vi "Autonomous Independent.vi"   [LabVIEW 2016]
doc: "This VI is called when autonomous begins, and will automatically be terminated when autonomous ends. You can carry out timed or sensor driven robot movement independently without needing to return to the caller."
uses:
  <vilib>/Rock Robotics/WPI/Ultrasonic/WPI_UltrasonicRangeUnits.ctl
  <vilib>/Rock Robotics/WPI/Utilities/WPI_GetSetVariantRefNum.vi
  <vilib>/Rock Robotics/Network Tables/NT Read String.vi
  <vilib>/Rock Robotics/Network Tables/NT Write Numeric Array.vi
  <vilib>/Rock Robotics/WPI/Ultrasonic/WPI_SonarSRF04DigitalRefNum Registry Get.vi
  <vilib>/Rock Robotics/WPI/Ultrasonic/WPI_SonarSRF04DigitalGetRange.vi
panel:
  # "Be sure to right-click and choose Data Operations>>Make Current Value default if you want to save the array values with the VI"
types:
  T1 = typedef "WPI_DriverStationPositionInfo.ctl" = enum16{"1", "2", "3"}
  T2 = typedef "WPI_JoystickDevRef.ctl" = cluster{"Device":T3}
  T3 = typedef "WPI_JoystickDeviceEnum.ctl" = enum16{"USB 0", "USB 1", "USB 2", "USB 3", "USB 4", "USB 5"}
  T4 = typedef "WPI_UltrasonicRangeUnits.ctl" = enum16{"inches", "mm"}
  T5 = typedef "WPI_EncoderDevRef.ctl" = cluster{"DevStatus":errorcluster, "EncoderIndex":T6, "CounterIndex":T7, "DistancePerCount":dbl, "Decoding Type":T8}
  T6 = typedef "FPGA_EncoderIdx.ctl" = enum8{"Enc 0", "Enc 1", "Enc 2", "Enc 3", "Enc 4", "Enc 5", "Enc 6", "Enc 7", "Invalid"}
  T7 = typedef "FPGA_CounterCtrSystemIndex.ctl" = enum8{"Ctr 0", "Ctr 1", "Ctr 2", "Ctr 3", "Ctr 4", "Ctr 5", "Ctr 6", "Ctr 7", "Invalid"}
  T8 = typedef "WPI_EncoderType.ctl" = enum16{"1x", "2x", "4x"}
  T9 = typedef "WPI_RobotDriveDevRef.ctl" = cluster{"DevStatus":errorcluster, "Motors[]":T10[], "Square Inputs":bool, "Max Output":dbl}
  T10 = typedef "WPI_MotorControlDeviceRef.ctl" = cluster{"DeviceStatus":errorcluster, "Type":T11, "PWM":cluster{"PWM Channel":T12, "DeadBand":T13}, "CAN":cluster{"Device Number":u8, "SetOutput VI Ref":variant, "GetOutput VI Ref":variant, "Enable VI Ref":variant, "Disable VI Ref":variant, "Data":variant}, "Invert":bool}
  T11 = typedef "WPI_MotorControlType.ctl" = enum16{"PWM", "CAN"}
  T12 = typedef "FPGA_DIOPWMChannel.ctl" = enum8{"PWM 0", "PWM 1", "PWM 2", "PWM 3", "PWM 4", "PWM 5", "PWM 6", "PWM 7", "PWM 8", "PWM 9", "PWM MXP 0", "PWM MXP 1", "PWM MXP 2", "PWM MXP 3", "PWM MXP 4", "PWM MXP 5", "PWM MXP 6", "PWM MXP 7", "PWM MXP 8", "PWM MXP 9", "Invalid"}
  T13 = typedef "WPI_PWMDeadband.ctl" = cluster{"Name":string, "maxPositivePwm":i32, "minPositivePwm":i32, "centerPwm":i32, "maxNegativePwm":i32, "minNegativePwm":i32, "angularRange":u16}
  T14 = typedef "Image Type" = u32
  T15 = typedef "WPI_CameraDevRef.ctl" = cluster{"Camera Address":string, "CameraStatus":errorcluster}
  T16 = typedef "WPI_CameraImageSize.ctl" = enum16{"640x480", "320x240", "160x120", "Custom"}
  T17 = typedef "IMAQ Image.ctl" = refnum<image>
  T18 = typedef "WPI_UltrasonicDeviceRef.ctl" = cluster{"DevStatus":errorcluster, "Ping Channel":T19, "Echo Channel":T19, "CntIndex":T7}
  T19 = typedef "FPGA_DIOChannel.ctl" = enum8{"DIO 0", "DIO 1", "DIO 2", "DIO 3", "DIO 4", "DIO 5", "DIO 6", "DIO 7", "DIO 8", "DIO 9", "DIO MXP 0", "DIO MXP 1", "DIO MXP 2", "DIO MXP 3", "DIO MXP 4", "DIO MXP 5", "DIO MXP 6", "DIO MXP 7", "DIO MXP 8", "DIO MXP 9", "DIO MXP 10", "DIO MXP 11", "DIO MXP 12", "DIO MXP 13", "DIO MXP 14", "DIO MXP 15", "SPI Port CS1", "SPI Port CS2", "SPI Port CS3", "SPI Port MISO", "SPI Port MOSI", "Invalid"}
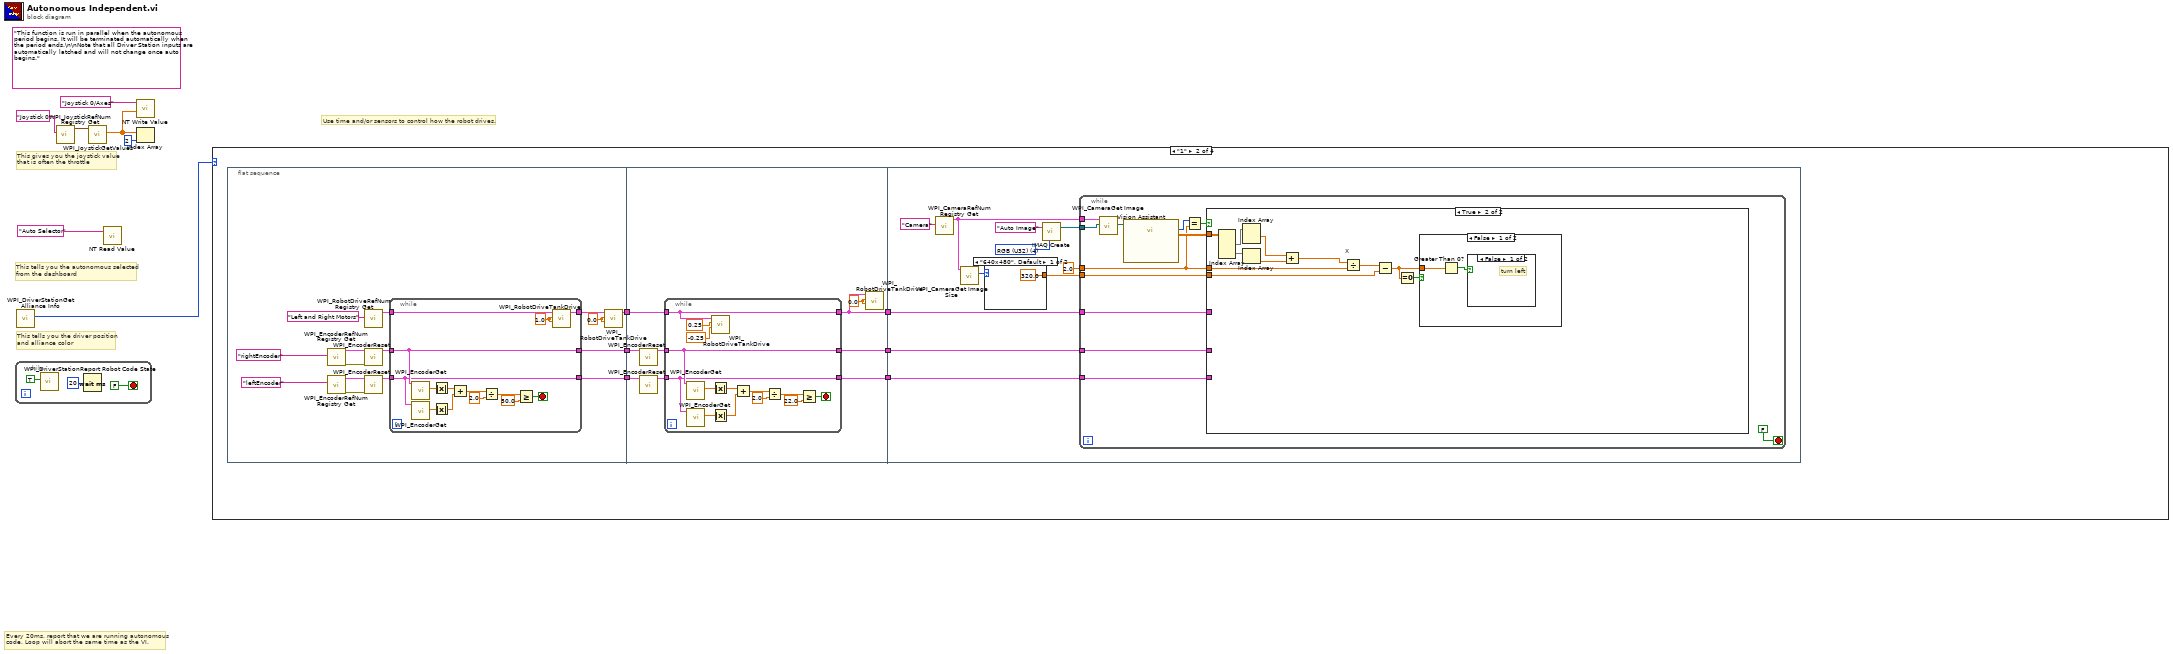
[diagram p0: block diagram]
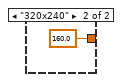
[diagram p3: hidden frame]
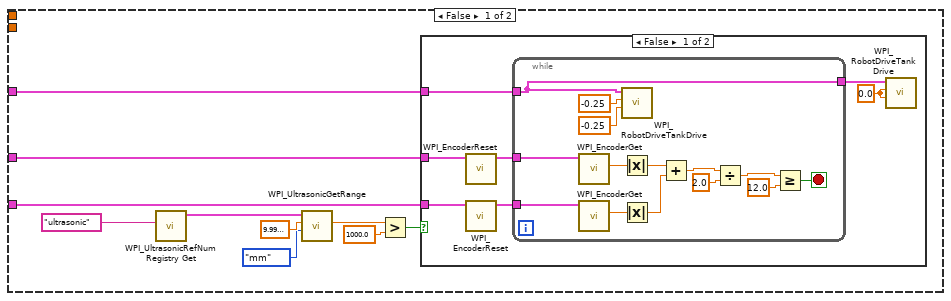
[diagram p4: hidden frame]
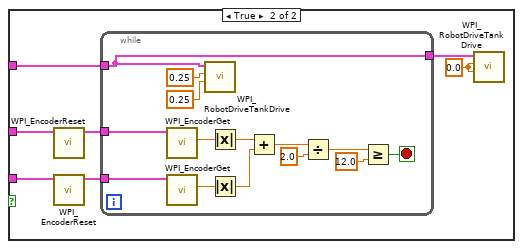
[diagram p5: hidden frame]
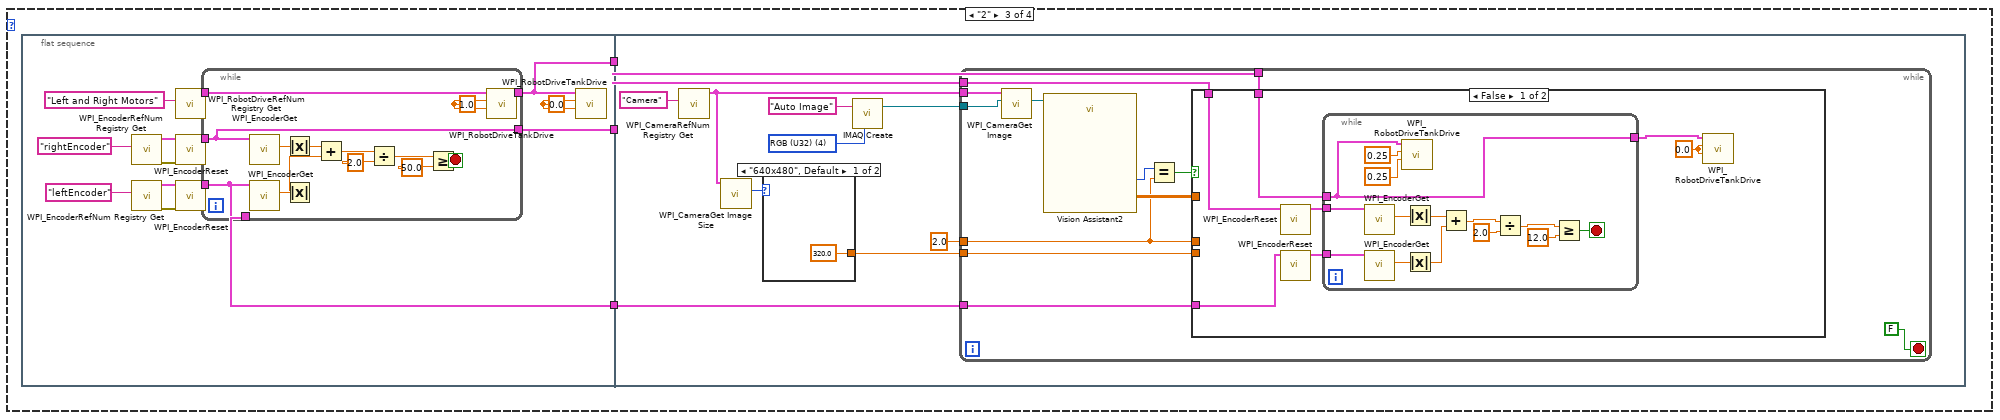
[diagram p8: hidden frame]
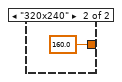
[diagram p9: hidden frame]
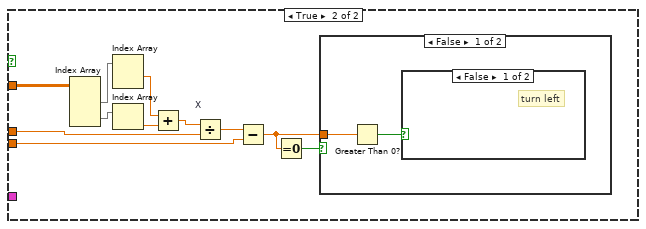
[diagram p10: hidden frame]
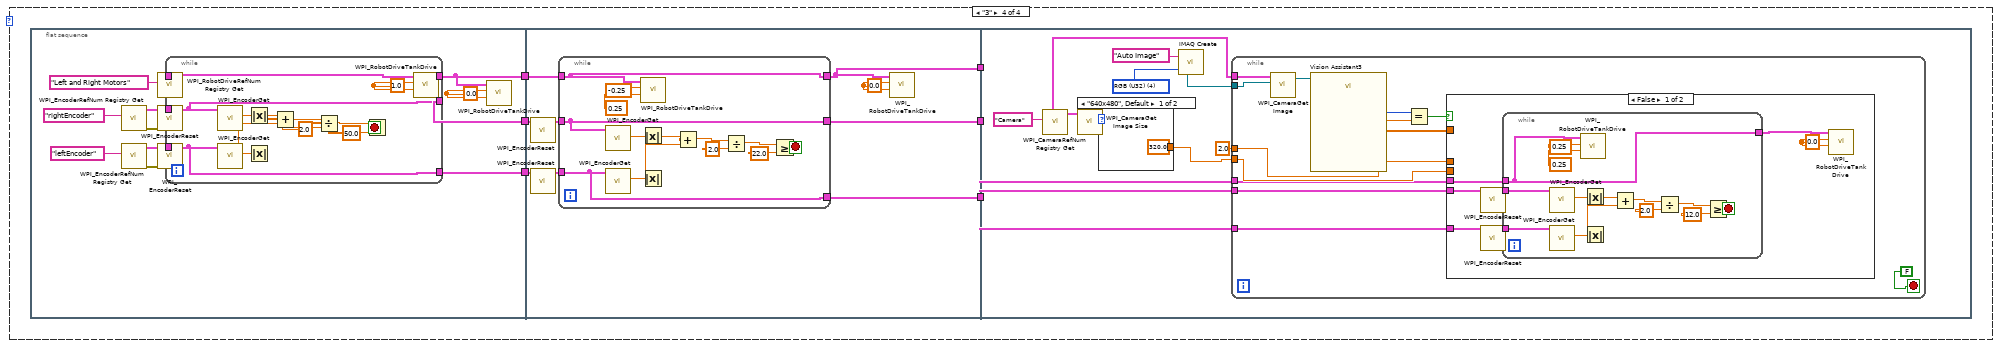
[diagram p13: hidden frame]
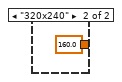
[diagram p14: hidden frame]
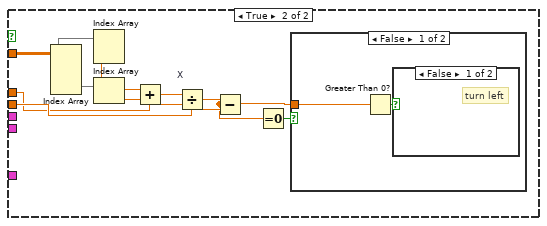
[diagram p15: hidden frame]
diagram:
  (unwired) "This function is run in parallel when the autonomous period begins. It will be terminated automatically when the period ends.\n\nNote that all Driver Station inputs are automatically latched and will not change once auto begins."
  # "This tells you the autonomous selected\nfrom the dashboard"
  # "Every 20ms, report that we are running autonomous\ncode. Loop will abort the same time as the VI."
  # "This gives you the joystick value\nthat is often the throttle"
  # "Use time and/or sensors to control how the robot drives."
  # "This tells you the driver position\nand alliance color"
  n1 = while {
    stop <- FALSE stop-if-true
    n2 = call <vilib>:"WPI_DriverStationReport Robot Code State.vi"("Autonomous"=TRUE) -> ()  [unwired: 10 in, 1 out]
    n3 = Wait (ms)(milliseconds to wait=u32 20) -> ()  [unwired: 1 out]
  }
  n4 = call <vilib>:"WPI_DriverStationGet Alliance Info.vi"() -> ("Position"=w1:T1)  [unwired: 11 out]
  n5 = call <vilib>:"WPI_JoystickRefNum Registry Get.vi"("refnum name"="Joystick 0") -> ("JoystickDevRef"=w6:T2)  [unwired: 1 in, 9 out]
  n6 = call <vilib>:"WPI_JoystickGetValues.vi"("JoystickDevRef"=w6) -> ("Axes"=w3:dbl[])  [unwired: 6 in, 4 out]
  n7 = call-poly <vilib>:"NT Read Value.vi"("Name"="Auto Selector") -> ()  [unwired: 9 in, 2 out]
  n8 = call-poly <vilib>:"NT Write Value.vi"("Numeric Array"=w3, "Name"="Joystick 0/Axes") -> ()  [unwired: 9 in, 1 out]
  n9 = Index Array(array=w3, index=2) -> ()  [unwired: 1 out]
  n10 = case shown="\"1\"" w1 {
    frame Default {
      # "You can put your main auto here, or you can right-click on the case and make any\nother frame be the default case."
      # "This is the frame that will execute if no selection is made, or if it is not recognized"
    }
    frame "1" {
      n11 = flat-sequence {
        tunnel: [w19] -> w16
        tunnel: [w18] -> w15
        tunnel: [w17] -> w14
        tunnel: w16 -> [w54]
        tunnel: w15 -> [w53]
        tunnel: w14 -> [w52]
        tunnel: [w48] -> w13
        tunnel: [w47] -> w12
        tunnel: [w46] -> w11
        tunnel: w13 -> [w71]
        tunnel: w12 -> [w70]
        tunnel: w11 -> [w69]
        frame #0 {
          w20 = 0.0 ("Left axis value")
          n12 = call <vilib>:"WPI_EncoderRefNum Registry Get.vi"("refnum name"="rightEncoder") -> ("error out"=w26:errorcluster, "EncoderDevRef"=w27:T5)  [unwired: 9 in]
          n13 = call <vilib>:"WPI_EncoderRefNum Registry Get.vi"("refnum name"="leftEncoder") -> ("error out"=w29:errorcluster, "EncoderDevRef"=w28:T5)  [unwired: 9 in]
          n14 = call <vilib>:"WPI_RobotDriveRefNum Registry Get.vi"("refnum name"="Left and Right Motors") -> ("RobotDriveDevRef"=w22:T9)  [unwired: 9 in, 1 out]
          n15 = call <vilib>:"WPI_EncoderReset.vi"("error in (no error)"=w26, "EncoderDevRef"=w27) -> ("EncoderDevRef"=w25:T5)  [unwired: 8 in, 1 out]
          n16 = call <vilib>:"WPI_EncoderReset.vi"("error in (no error)"=w29, "EncoderDevRef"=w28) -> ("EncoderDevRef"=w24:T5)  [unwired: 8 in, 1 out]
          n17 = while {
            tunnel: w25 -> [w33]
            tunnel: w24 -> [w32]
            tunnel: w22 -> [w37]
            tunnel: [w35] -> w21
            tunnel: [w33] -> w18
            tunnel: [w32] -> w17
            stop <- w34 stop-if-true
            w36 = 1.0 ("Left axis value")
            n18 = call <vilib>:"WPI_EncoderGet.vi"("EncoderDevRef"=w33) -> ("Distance"=w45:dbl)  [unwired: 5 in, 5 out]
            n19 = call <vilib>:"WPI_EncoderGet.vi"("EncoderDevRef"=w32) -> ("Distance"=w44:dbl)  [unwired: 5 in, 5 out]
            n20 = Absolute Value(x=w45) -> (abs(x)=w42:dbl)
            n21 = Absolute Value(x=w44) -> (abs(x)=w43:dbl)
            n22 = Add(x=w42, y=w43) -> (x+y=w41:dbl)
            n23 = Divide(x=w41, y=2.0) -> (x/y=w39:dbl)
            n24 = Greater Or Equal?(x=w39, y=50.0) -> (x >= y?=w34:bool)
            n25 = call <vilib>:"WPI_RobotDriveTankDrive.vi"("Right axis value"=w36, "Left axis value"=w36, "RobotDriveDevRef"=w37) -> ("RobotDriveDevRef"=w35:T9)  [unwired: 6 in, 2 out]
          }
          n26 = call <vilib>:"WPI_RobotDriveTankDrive.vi"("Right axis value"=w20, "Left axis value"=w20, "RobotDriveDevRef"=w21) -> ("RobotDriveDevRef"=w19:T9)  [unwired: 6 in, 2 out]
        }
        frame #1 {
          w49 = 0.0 ("Left axis value")
          n27 = call <vilib>:"WPI_EncoderReset.vi"("EncoderDevRef"=w53) -> ("EncoderDevRef"=w51:T5)  [unwired: 9 in, 1 out]
          n28 = call <vilib>:"WPI_EncoderReset.vi"("EncoderDevRef"=w52) -> ("EncoderDevRef"=w50:T5)  [unwired: 9 in, 1 out]
          n29 = while {
            tunnel: w54 -> [w57]
            tunnel: w51 -> [w56]
            tunnel: w50 -> [w55]
            tunnel: [w57] -> w48
            tunnel: [w56] -> w47
            tunnel: [w55] -> w46
            stop <- w58 stop-if-true
            n30 = call <vilib>:"WPI_EncoderGet.vi"("EncoderDevRef"=w56) -> ("Distance"=w66:dbl)  [unwired: 5 in, 5 out]
            n31 = call <vilib>:"WPI_EncoderGet.vi"("EncoderDevRef"=w55) -> ("Distance"=w65:dbl)  [unwired: 5 in, 5 out]
            n32 = call <vilib>:"WPI_RobotDriveTankDrive.vi"("Right axis value"=-0.25, "Left axis value"=0.25, "RobotDriveDevRef"=w57) -> ()  [unwired: 6 in, 3 out]
            n33 = Absolute Value(x=w66) -> (abs(x)=w64:dbl)
            n34 = Absolute Value(x=w65) -> (abs(x)=w63:dbl)
            n35 = Add(x=w64, y=w63) -> (x+y=w62:dbl)
            n36 = Divide(x=w62, y=2.0) -> (x/y=w60:dbl)
            n37 = Greater Or Equal?(x=w60, y=22.0) -> (x >= y?=w58:bool)
          }
          n38 = call <vilib>:"WPI_RobotDriveTankDrive.vi"("Right axis value"=w49, "Left axis value"=w49, "RobotDriveDevRef"=w48) -> ()  [unwired: 6 in, 3 out]
        }
        frame #2 {
          w78 = T14 4 items=["Grayscale (U8)", "Grayscale (I16)", "Grayscale (SGL)", "Complex (CSG)", "RGB (U32)", "HSL (U32)", "RGB (U64)"] ("Image Type")
          n39 = call <vilib>:"WPI_CameraRefNum Registry Get.vi"("refnum name"="Camera") -> ("CameraDevRef"=w73:T15)  [unwired: 9 in, 1 out]
          n40 = call <vilib>:"WPI_CameraGet Image Size.vi"("CameraDevRef"=w73) -> ("Image Size"=w72:T16)  [unwired: 7 in, 3 out]
          n41 = case shown="\"640x480\", Default" w72 {
            tunnel: [320.0 160.0] -> w75
            frame "640x480", Default {
            }
            frame "320x240" {
            }
          }
          n42 = call "IMAQ Create"("Image Name"="Auto Image", "Image Type"=w78) -> ("New Image"=w76:T17)  [unwired: 2 in, 2 out]
          n43 = while {
            tunnel: w73 -> [w93]
            tunnel: w76 -> [w92]
            tunnel: 2.0 -> [w85]
            tunnel: w75 -> [w86]
            tunnel: w71 -> [w84]
            tunnel: w70 -> [w83]
            tunnel: w69 -> [w82]
            stop <- FALSE stop-if-true
            n44 = call <vilib>:"WPI_CameraGet Image.vi"("Image"=w92, "CameraDevRef"=w93) -> ("Image Out"=w91:T17)  [unwired: 7 in, 2 out]
            n45 = call "Vision Assistant"("Image In"=w91) -> ("Number of Particles (Particle Analysis 1)"=w89:i32, "Particle Measurements (Pixels) (Particle Analysis 1)"=w87:dbl[][])  [unwired: 22 in, 3 out]
            n46 = Equal?(x=w89, y=w85) -> (x = y?=w88:bool)
            n47 = case shown="True" w88 {
              tunnel: w87 -> [_ w149]
              tunnel: w86 -> [_ w148]
              tunnel: w85 -> [_ w147]
              tunnel: w84 -> [w96 _]
              tunnel: w83 -> [w95 _]
              tunnel: w82 -> [w94 _]
              frame False {
                n48 = call-poly <vilib>:"WPI_UltrasonicRefNum Registry Get.vi"("refnum name"="ultrasonic") -> ("SonarSRF04DevRef"=w102:T18)  [unwired: 9 in, 1 out]
                n49 = call-poly <vilib>:"WPI_UltrasonicGetRange.vi"("Range Units"=WPI_UltrasonicRangeUnits."mm", "ping time (s)"=sgl 1e-05, "SonarSRF04DevRef"=w102) -> ("Distance"=w99:dbl)  [unwired: 6 in, 2 out]
                n50 = Greater?(x=w99, y=1000.0) -> (0:w97:bool)
                n51 = case shown="False" w97 {
                  tunnel: w96 -> [w106 w127]
                  tunnel: w95 -> [w105 w126]
                  tunnel: w94 -> [w104 w125]
                  frame False {
                    w107 = 0.0 ("Left axis value")
                    n52 = call <vilib>:"WPI_EncoderReset.vi"("EncoderDevRef"=w105) -> ("EncoderDevRef"=w110:T5)  [unwired: 9 in, 1 out]
                    n53 = call <vilib>:"WPI_EncoderReset.vi"("EncoderDevRef"=w104) -> ("EncoderDevRef"=w109:T5)  [unwired: 9 in, 1 out]
                    n54 = while {
                      tunnel: w106 -> [w111]
                      tunnel: w110 -> [w122]
                      tunnel: w109 -> [w121]
                      tunnel: [w111] -> w108
                      stop <- w112 stop-if-true
                      n55 = call <vilib>:"WPI_EncoderGet.vi"("EncoderDevRef"=w122) -> ("Distance"=w120:dbl)  [unwired: 5 in, 5 out]
                      n56 = call <vilib>:"WPI_EncoderGet.vi"("EncoderDevRef"=w121) -> ("Distance"=w119:dbl)  [unwired: 5 in, 5 out]
                      n57 = call <vilib>:"WPI_RobotDriveTankDrive.vi"("Right axis value"=-0.25, "Left axis value"=-0.25, "RobotDriveDevRef"=w111) -> ()  [unwired: 6 in, 3 out]
                      n58 = Absolute Value(x=w120) -> (abs(x)=w118:dbl)
                      n59 = Absolute Value(x=w119) -> (abs(x)=w117:dbl)
                      n60 = Add(x=w118, y=w117) -> (x+y=w116:dbl)
                      n61 = Divide(x=w116, y=2.0) -> (x/y=w114:dbl)
                      n62 = Greater Or Equal?(x=w114, y=12.0) -> (x >= y?=w112:bool)
                    }
                    n63 = call <vilib>:"WPI_RobotDriveTankDrive.vi"("Right axis value"=w107, "Left axis value"=w107, "RobotDriveDevRef"=w108) -> ()  [unwired: 6 in, 3 out]
                  }
                  frame True {
                    w128 = 0.0 ("Left axis value")
                    n64 = call <vilib>:"WPI_EncoderReset.vi"("EncoderDevRef"=w126) -> ("EncoderDevRef"=w131:T5)  [unwired: 9 in, 1 out]
                    n65 = call <vilib>:"WPI_EncoderReset.vi"("EncoderDevRef"=w125) -> ("EncoderDevRef"=w130:T5)  [unwired: 9 in, 1 out]
                    n66 = while {
                      tunnel: w127 -> [w132]
                      tunnel: w131 -> [w143]
                      tunnel: w130 -> [w142]
                      tunnel: [w132] -> w129
                      stop <- w133 stop-if-true
                      n67 = call <vilib>:"WPI_EncoderGet.vi"("EncoderDevRef"=w143) -> ("Distance"=w141:dbl)  [unwired: 5 in, 5 out]
                      n68 = call <vilib>:"WPI_EncoderGet.vi"("EncoderDevRef"=w142) -> ("Distance"=w140:dbl)  [unwired: 5 in, 5 out]
                      n69 = call <vilib>:"WPI_RobotDriveTankDrive.vi"("Right axis value"=0.25, "Left axis value"=0.25, "RobotDriveDevRef"=w132) -> ()  [unwired: 6 in, 3 out]
                      n70 = Absolute Value(x=w141) -> (abs(x)=w139:dbl)
                      n71 = Absolute Value(x=w140) -> (abs(x)=w138:dbl)
                      n72 = Add(x=w139, y=w138) -> (x+y=w137:dbl)
                      n73 = Divide(x=w137, y=2.0) -> (x/y=w135:dbl)
                      n74 = Greater Or Equal?(x=w135, y=12.0) -> (x >= y?=w133:bool)
                    }
                    n75 = call <vilib>:"WPI_RobotDriveTankDrive.vi"("Right axis value"=w128, "Left axis value"=w128, "RobotDriveDevRef"=w129) -> ()  [unwired: 6 in, 3 out]
                  }
                }
              }
              frame True {
                n76 = Index Array(array=w149) -> (element #1=w150:dbl[], element #2=w151:dbl[])  [unwired: 4 in]
                n77 = Index Array(array=w150) -> (element #1=w152:dbl)  [unwired: 2 in, 1 out]
                n78 = Index Array(array=w151) -> (element=w153:dbl)  [unwired: 1 in]
                n79 = Add(x=w152, y=w153) -> (x+y=w154:dbl)
                n80 = Divide "X"(x=w154, y=w147) -> (x/y=w155:dbl)
                n81 = Subtract(x=w155, y=w148) -> (x-y=w146:dbl)
                n82 = Equal To 0?(x=w146) -> (x = 0?=w156:bool)
                n83 = case shown="False" w156 {
                  tunnel: w146 -> [w158 _]
                  frame False {
                    n84 = Greater Than 0?(x=w158) -> (x > 0?=w157:bool)
                    n85 = case shown="False" w157 {
                      frame False {
                        # "turn left"
                      }
                      frame True {
                        # "turn right"
                      }
                    }
                  }
                  frame True {
                    # "Drive forwards"
                  }
                }
              }
            }
          }
        }
      }
    }
    frame "2" {
      n86 = flat-sequence {
        tunnel: [w164] -> w161
        tunnel: [w163] -> w160
        tunnel: [w162] -> w159
        tunnel: w161 -> [w192]
        tunnel: w160 -> [w191]
        tunnel: w159 -> [w190]
        frame #0 {
          w165 = 0.0 ("Left axis value")
          n87 = call <vilib>:"WPI_EncoderRefNum Registry Get.vi"("refnum name"="rightEncoder") -> ("error out"=w170:errorcluster, "EncoderDevRef"=w171:T5)  [unwired: 9 in]
          n88 = call <vilib>:"WPI_EncoderRefNum Registry Get.vi"("refnum name"="leftEncoder") -> ("error out"=w173:errorcluster, "EncoderDevRef"=w172:T5)  [unwired: 9 in]
          n89 = call <vilib>:"WPI_RobotDriveRefNum Registry Get.vi"("refnum name"="Left and Right Motors") -> ("RobotDriveDevRef"=w166:T9)  [unwired: 9 in, 1 out]
          n90 = call <vilib>:"WPI_EncoderReset.vi"("error in (no error)"=w170, "EncoderDevRef"=w171) -> ("EncoderDevRef"=w169:T5)  [unwired: 8 in, 1 out]
          n91 = call <vilib>:"WPI_EncoderReset.vi"("error in (no error)"=w173, "EncoderDevRef"=w172) -> ("EncoderDevRef"=w168:T5)  [unwired: 8 in, 1 out]
          n92 = while {
            tunnel: w169 -> [w177]
            tunnel: w168 -> [w176]
            tunnel: w166 -> [w181]
            tunnel: [w179] -> w164
            tunnel: [w177] -> w163
            tunnel: [w176] -> w162
            stop <- w178 stop-if-true
            w180 = 1.0 ("Left axis value")
            n93 = call <vilib>:"WPI_EncoderGet.vi"("EncoderDevRef"=w177) -> ("Distance"=w189:dbl)  [unwired: 5 in, 5 out]
            n94 = call <vilib>:"WPI_EncoderGet.vi"("EncoderDevRef"=w176) -> ("Distance"=w188:dbl)  [unwired: 5 in, 5 out]
            n95 = Absolute Value(x=w189) -> (abs(x)=w186:dbl)
            n96 = Absolute Value(x=w188) -> (abs(x)=w187:dbl)
            n97 = Add(x=w186, y=w187) -> (x+y=w185:dbl)
            n98 = Divide(x=w185, y=2.0) -> (x/y=w183:dbl)
            n99 = Greater Or Equal?(x=w183, y=50.0) -> (x >= y?=w178:bool)
            n100 = call <vilib>:"WPI_RobotDriveTankDrive.vi"("Right axis value"=w180, "Left axis value"=w180, "RobotDriveDevRef"=w181) -> ("RobotDriveDevRef"=w179:T9)  [unwired: 6 in, 2 out]
          }
          n101 = call <vilib>:"WPI_RobotDriveTankDrive.vi"("Right axis value"=w165, "Left axis value"=w165, "RobotDriveDevRef"=w164) -> ()  [unwired: 6 in, 3 out]
        }
        frame #1 {
          w199 = T14 4 items=["Grayscale (U8)", "Grayscale (I16)", "Grayscale (SGL)", "Complex (CSG)", "RGB (U32)", "HSL (U32)", "RGB (U64)"] ("Image Type")
          n102 = call <vilib>:"WPI_CameraRefNum Registry Get.vi"("refnum name"="Camera") -> ("CameraDevRef"=w194:T15)  [unwired: 9 in, 1 out]
          n103 = call <vilib>:"WPI_CameraGet Image Size.vi"("CameraDevRef"=w194) -> ("Image Size"=w193:T16)  [unwired: 7 in, 3 out]
          n104 = case shown="\"640x480\", Default" w193 {
            tunnel: [320.0 160.0] -> w196
            frame "640x480", Default {
            }
            frame "320x240" {
            }
          }
          n105 = call "IMAQ Create"("Image Name"="Auto Image", "Image Type"=w199) -> ("New Image"=w197:T17)  [unwired: 2 in, 2 out]
          n106 = while {
            tunnel: w194 -> [w214]
            tunnel: w197 -> [w213]
            tunnel: 2.0 -> [w206]
            tunnel: w196 -> [w207]
            tunnel: w192 -> [w205]
            tunnel: w191 -> [w204]
            tunnel: w190 -> [w203]
            stop <- FALSE stop-if-true
            n107 = call <vilib>:"WPI_CameraGet Image.vi"("Image"=w213, "CameraDevRef"=w214) -> ("Image Out"=w212:T17)  [unwired: 7 in, 2 out]
            n108 = call "Vision Assistant2"("Image In"=w212) -> ("Number of Particles (Particle Analysis 1)"=w210:i32, "Particle Measurements (Pixels) (Particle Analysis 1)"=w208:dbl[][])  [unwired: 22 in, 3 out]
            n109 = Equal?(x=w210, y=w206) -> (x = y?=w209:bool)
            n110 = case shown="False" w209 {
              tunnel: w208 -> [_ w239]
              tunnel: w207 -> [_ w238]
              tunnel: w206 -> [_ w237]
              tunnel: w205 -> [w217 _]
              tunnel: w204 -> [w216 _]
              tunnel: w203 -> [w215 _]
              frame False {
                w218 = 0.0 ("Left axis value")
                n111 = call <vilib>:"WPI_EncoderReset.vi"("EncoderDevRef"=w216) -> ("EncoderDevRef"=w221:T5)  [unwired: 9 in, 1 out]
                n112 = call <vilib>:"WPI_EncoderReset.vi"("EncoderDevRef"=w215) -> ("EncoderDevRef"=w220:T5)  [unwired: 9 in, 1 out]
                n113 = while {
                  tunnel: w217 -> [w222]
                  tunnel: w221 -> [w233]
                  tunnel: w220 -> [w232]
                  tunnel: [w222] -> w219
                  stop <- w223 stop-if-true
                  n114 = call <vilib>:"WPI_EncoderGet.vi"("EncoderDevRef"=w233) -> ("Distance"=w231:dbl)  [unwired: 5 in, 5 out]
                  n115 = call <vilib>:"WPI_EncoderGet.vi"("EncoderDevRef"=w232) -> ("Distance"=w230:dbl)  [unwired: 5 in, 5 out]
                  n116 = call <vilib>:"WPI_RobotDriveTankDrive.vi"("Right axis value"=0.25, "Left axis value"=0.25, "RobotDriveDevRef"=w222) -> ()  [unwired: 6 in, 3 out]
                  n117 = Absolute Value(x=w231) -> (abs(x)=w229:dbl)
                  n118 = Absolute Value(x=w230) -> (abs(x)=w228:dbl)
                  n119 = Add(x=w229, y=w228) -> (x+y=w227:dbl)
                  n120 = Divide(x=w227, y=2.0) -> (x/y=w225:dbl)
                  n121 = Greater Or Equal?(x=w225, y=12.0) -> (x >= y?=w223:bool)
                }
                n122 = call <vilib>:"WPI_RobotDriveTankDrive.vi"("Right axis value"=w218, "Left axis value"=w218, "RobotDriveDevRef"=w219) -> ()  [unwired: 6 in, 3 out]
              }
              frame True {
                n123 = Index Array(array=w239) -> (element #1=w240:dbl[], element #2=w241:dbl[])  [unwired: 4 in]
                n124 = Index Array(array=w240) -> (element #1=w242:dbl)  [unwired: 2 in, 1 out]
                n125 = Index Array(array=w241) -> (element=w243:dbl)  [unwired: 1 in]
                n126 = Add(x=w242, y=w243) -> (x+y=w244:dbl)
                n127 = Divide "X"(x=w244, y=w237) -> (x/y=w245:dbl)
                n128 = Subtract(x=w245, y=w238) -> (x-y=w236:dbl)
                n129 = Equal To 0?(x=w236) -> (x = 0?=w246:bool)
                n130 = case shown="False" w246 {
                  tunnel: w236 -> [w248 _]
                  frame False {
                    n131 = Greater Than 0?(x=w248) -> (x > 0?=w247:bool)
                    n132 = case shown="False" w247 {
                      frame False {
                        # "turn left"
                      }
                      frame True {
                        # "turn right"
                      }
                    }
                  }
                  frame True {
                    # "Drive forwards"
                  }
                }
              }
            }
          }
        }
      }
    }
    frame "3" {
      n133 = flat-sequence {
        tunnel: [w257] -> w254
        tunnel: [w256] -> w253
        tunnel: [w255] -> w252
        tunnel: w254 -> [w289]
        tunnel: w253 -> [w288]
        tunnel: w252 -> [w287]
        tunnel: [w285] -> w251
        tunnel: [w284] -> w250
        tunnel: [w283] -> w249
        tunnel: w251 -> [w308]
        tunnel: w250 -> [w307]
        tunnel: w249 -> [w306]
        frame #0 {
          w258 = 0.0 ("Left axis value")
          n134 = call <vilib>:"WPI_EncoderRefNum Registry Get.vi"("refnum name"="rightEncoder") -> ("error out"=w263:errorcluster, "EncoderDevRef"=w264:T5)  [unwired: 9 in]
          n135 = call <vilib>:"WPI_EncoderRefNum Registry Get.vi"("refnum name"="leftEncoder") -> ("error out"=w266:errorcluster, "EncoderDevRef"=w265:T5)  [unwired: 9 in]
          n136 = call <vilib>:"WPI_RobotDriveRefNum Registry Get.vi"("refnum name"="Left and Right Motors") -> ("RobotDriveDevRef"=w259:T9)  [unwired: 9 in, 1 out]
          n137 = call <vilib>:"WPI_EncoderReset.vi"("error in (no error)"=w263, "EncoderDevRef"=w264) -> ("EncoderDevRef"=w262:T5)  [unwired: 8 in, 1 out]
          n138 = call <vilib>:"WPI_EncoderReset.vi"("error in (no error)"=w266, "EncoderDevRef"=w265) -> ("EncoderDevRef"=w261:T5)  [unwired: 8 in, 1 out]
          n139 = while {
            tunnel: w262 -> [w270]
            tunnel: w261 -> [w269]
            tunnel: w259 -> [w274]
            tunnel: [w272] -> w257
            tunnel: [w270] -> w256
            tunnel: [w269] -> w255
            stop <- w271 stop-if-true
            w273 = 1.0 ("Left axis value")
            n140 = call <vilib>:"WPI_EncoderGet.vi"("EncoderDevRef"=w270) -> ("Distance"=w282:dbl)  [unwired: 5 in, 5 out]
            n141 = call <vilib>:"WPI_EncoderGet.vi"("EncoderDevRef"=w269) -> ("Distance"=w281:dbl)  [unwired: 5 in, 5 out]
            n142 = Absolute Value(x=w282) -> (abs(x)=w279:dbl)
            n143 = Absolute Value(x=w281) -> (abs(x)=w280:dbl)
            n144 = Add(x=w279, y=w280) -> (x+y=w278:dbl)
            n145 = Divide(x=w278, y=2.0) -> (x/y=w276:dbl)
            n146 = Greater Or Equal?(x=w276, y=50.0) -> (x >= y?=w271:bool)
            n147 = call <vilib>:"WPI_RobotDriveTankDrive.vi"("Right axis value"=w273, "Left axis value"=w273, "RobotDriveDevRef"=w274) -> ("RobotDriveDevRef"=w272:T9)  [unwired: 6 in, 2 out]
          }
          n148 = call <vilib>:"WPI_RobotDriveTankDrive.vi"("Right axis value"=w258, "Left axis value"=w258, "RobotDriveDevRef"=w257) -> ()  [unwired: 6 in, 3 out]
        }
        frame #1 {
          w286 = 0.0 ("Left axis value")
          n149 = call <vilib>:"WPI_EncoderReset.vi"("EncoderDevRef"=w288) -> ("EncoderDevRef"=w291:T5)  [unwired: 9 in, 1 out]
          n150 = call <vilib>:"WPI_EncoderReset.vi"("EncoderDevRef"=w287) -> ("EncoderDevRef"=w290:T5)  [unwired: 9 in, 1 out]
          n151 = while {
            tunnel: w289 -> [w294]
            tunnel: w291 -> [w292]
            tunnel: w290 -> [w293]
            tunnel: [w294] -> w285
            tunnel: [w293] -> w284
            tunnel: [w292] -> w283
            stop <- w295 stop-if-true
            n152 = call <vilib>:"WPI_EncoderGet.vi"("EncoderDevRef"=w292) -> ("Distance"=w303:dbl)  [unwired: 5 in, 5 out]
            n153 = call <vilib>:"WPI_EncoderGet.vi"("EncoderDevRef"=w293) -> ("Distance"=w302:dbl)  [unwired: 5 in, 5 out]
            n154 = call <vilib>:"WPI_RobotDriveTankDrive.vi"("Right axis value"=0.25, "Left axis value"=-0.25, "RobotDriveDevRef"=w294) -> ()  [unwired: 6 in, 3 out]
            n155 = Absolute Value(x=w303) -> (abs(x)=w301:dbl)
            n156 = Absolute Value(x=w302) -> (abs(x)=w300:dbl)
            n157 = Add(x=w301, y=w300) -> (x+y=w299:dbl)
            n158 = Divide(x=w299, y=2.0) -> (x/y=w297:dbl)
            n159 = Greater Or Equal?(x=w297, y=22.0) -> (x >= y?=w295:bool)
          }
          n160 = call <vilib>:"WPI_RobotDriveTankDrive.vi"("Right axis value"=w286, "Left axis value"=w286, "RobotDriveDevRef"=w285) -> ()  [unwired: 6 in, 3 out]
        }
        frame #2 {
          w315 = T14 4 items=["Grayscale (U8)", "Grayscale (I16)", "Grayscale (SGL)", "Complex (CSG)", "RGB (U32)", "HSL (U32)", "RGB (U64)"] ("Image Type")
          n161 = call <vilib>:"WPI_CameraRefNum Registry Get.vi"("refnum name"="Camera") -> ("CameraDevRef"=w310:T15)  [unwired: 9 in, 1 out]
          n162 = call <vilib>:"WPI_CameraGet Image Size.vi"("CameraDevRef"=w310) -> ("Image Size"=w309:T16)  [unwired: 7 in, 3 out]
          n163 = case shown="\"640x480\", Default" w309 {
            tunnel: [320.0 160.0] -> w312
            frame "640x480", Default {
            }
            frame "320x240" {
            }
          }
          n164 = call "IMAQ Create"("Image Name"="Auto Image", "Image Type"=w315) -> ("New Image"=w313:T17)  [unwired: 2 in, 2 out]
          n165 = while {
            tunnel: w310 -> [w330]
            tunnel: w313 -> [w329]
            tunnel: 2.0 -> [w322]
            tunnel: w312 -> [w323]
            tunnel: w308 -> [w321]
            tunnel: w307 -> [w320]
            tunnel: w306 -> [w319]
            stop <- FALSE stop-if-true
            n166 = call <vilib>:"WPI_CameraGet Image.vi"("Image"=w329, "CameraDevRef"=w330) -> ("Image Out"=w328:T17)  [unwired: 7 in, 2 out]
            n167 = call "Vision Assistant3"("Image In"=w328) -> ("Number of Particles (Particle Analysis 1)"=w326:i32, "Particle Measurements (Pixels) (Particle Analysis 1)"=w324:dbl[][])  [unwired: 22 in, 3 out]
            n168 = Equal?(x=w326, y=w322) -> (x = y?=w325:bool)
            n169 = case shown="False" w325 {
              tunnel: w324 -> [_ w355]
              tunnel: w323 -> [_ w354]
              tunnel: w322 -> [_ w353]
              tunnel: w321 -> [w333 _]
              tunnel: w320 -> [w331 _]
              tunnel: w319 -> [w332 _]
              frame False {
                w334 = 0.0 ("Left axis value")
                n170 = call <vilib>:"WPI_EncoderReset.vi"("EncoderDevRef"=w332) -> ("EncoderDevRef"=w337:T5)  [unwired: 9 in, 1 out]
                n171 = call <vilib>:"WPI_EncoderReset.vi"("EncoderDevRef"=w331) -> ("EncoderDevRef"=w336:T5)  [unwired: 9 in, 1 out]
                n172 = while {
                  tunnel: w333 -> [w338]
                  tunnel: w337 -> [w349]
                  tunnel: w336 -> [w348]
                  tunnel: [w338] -> w335
                  stop <- w339 stop-if-true
                  n173 = call <vilib>:"WPI_EncoderGet.vi"("EncoderDevRef"=w349) -> ("Distance"=w347:dbl)  [unwired: 5 in, 5 out]
                  n174 = call <vilib>:"WPI_EncoderGet.vi"("EncoderDevRef"=w348) -> ("Distance"=w346:dbl)  [unwired: 5 in, 5 out]
                  n175 = call <vilib>:"WPI_RobotDriveTankDrive.vi"("Right axis value"=0.25, "Left axis value"=0.25, "RobotDriveDevRef"=w338) -> ()  [unwired: 6 in, 3 out]
                  n176 = Absolute Value(x=w347) -> (abs(x)=w345:dbl)
                  n177 = Absolute Value(x=w346) -> (abs(x)=w344:dbl)
                  n178 = Add(x=w345, y=w344) -> (x+y=w343:dbl)
                  n179 = Divide(x=w343, y=2.0) -> (x/y=w341:dbl)
                  n180 = Greater Or Equal?(x=w341, y=12.0) -> (x >= y?=w339:bool)
                }
                n181 = call <vilib>:"WPI_RobotDriveTankDrive.vi"("Right axis value"=w334, "Left axis value"=w334, "RobotDriveDevRef"=w335) -> ()  [unwired: 6 in, 3 out]
              }
              frame True {
                n182 = Index Array(array=w355) -> (element #1=w356:dbl[], element #2=w357:dbl[])  [unwired: 4 in]
                n183 = Index Array(array=w356) -> (element #1=w358:dbl)  [unwired: 2 in, 1 out]
                n184 = Index Array(array=w357) -> (element=w359:dbl)  [unwired: 1 in]
                n185 = Add(x=w358, y=w359) -> (x+y=w360:dbl)
                n186 = Divide "X"(x=w360, y=w353) -> (x/y=w361:dbl)
                n187 = Subtract(x=w361, y=w354) -> (x-y=w352:dbl)
                n188 = Equal To 0?(x=w352) -> (x = 0?=w362:bool)
                n189 = case shown="False" w362 {
                  tunnel: w352 -> [w364 _]
                  frame False {
                    n190 = Greater Than 0?(x=w364) -> (x > 0?=w363:bool)
                    n191 = case shown="False" w363 {
                      frame False {
                        # "turn left"
                      }
                      frame True {
                        # "turn right"
                      }
                    }
                  }
                  frame True {
                    # "Drive forwards"
                  }
                }
              }
            }
          }
        }
      }
    }
  }
